vi "test_error_handling.vi"(8 "error in":errorcluster) -> (0 "error out":errorcluster)   [LabVIEW 2020, in "Conformance MCP Server.lvlib"]
doc: "Conformance fixture (scenario tools-call-error). Takes no arguments and always fails: error out carries error 5000 with the text \"This tool intentionally returns an error for testing\", so the server answers tools/call with isError true."
uses:
  Conformance MCP Server.lvlib
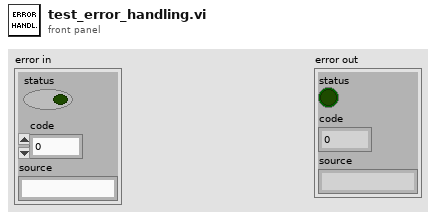
[diagram p1: front panel]
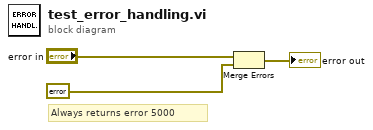
[diagram p0: block diagram]
diagram:
  # "Always returns error 5000"
  n1 = Merge Errors("error in", errorcluster {"status"=TRUE, "code"=5000, "source"="This tool intentionally returns an error for testing"} ("error")) -> (→"error out":errorcluster)
